vi "Check Modern MCP Request.vi"(7 "Mcp-Name":string, 8 "error in":errorcluster, 9 "Mcp-Method":string, 10 "protocol version":string, 11 "MCP Request Metadata":T1) -> (0 "error out":errorcluster, 1 "response":string, 2 "status code":u16, 3 "refused":bool)   [LabVIEW 2020, in "MCP Server.lvlib"]
doc: "Checks a request against the rules of MCP 2026-07-28 before it is handled, and says whether it is refused, with which HTTP status and which JSON-RPC error body. A legacy request is never refused here, except a JSON array that comes with modern headers.\n\nChecked in this order, the first failing check wins:\n- MCP-Protocol-Version header missing or different from the _meta protocolVersion: 400, -32020 (header mismatch).\n- protocolVersion not one of the modern versions of Supported Protocol Versions.vi: 400, -32022 with data.supported and data.requested.\n- Mcp-Method header missing or different from method: 400, -32020.\n- tools/call and prompts/get: Mcp-Name must equal params.name; resources/read: params.uri. A value =?base64?...?= is decoded first. Missing or different: 400, -32020.\n- io.modelcontextprotocol/clientCapabilities missing in params._meta: 400, -32602.\n- A method the modern era does not have (it has server/discover, tools/list, tools/call, prompts/list, prompts/get, resources/list, resources/read and resources/templates/list): 404, -32601. Notifications (no id) are not refused for this.\nA JSON array (batch) that comes with modern headers (an Mcp-Method header, or a modern MCP-Protocol-Version) is refused with 400, -32600.\n\nThe JSONtext errors are merged and cleared here. error in is passed through unchanged and does not stop the checks."
uses:
  MCP Server.lvlib
  5a72b263-2192-4f58-90a6-a4dd77c4a3e2.vi
  dc7c98e2-eea7-441a-9c60-934f37bda1c1.vi
  1b19c665-3783-46bd-b4e4-7a0e92e2d9d1.vi
  <vilib>/JDP Science/JSONtext/Variant to JSON Text.vi
  <vilib>/JDP Science/JSONtext/LVClass Serializer/JSONtext LVClass Serializer.lvclass
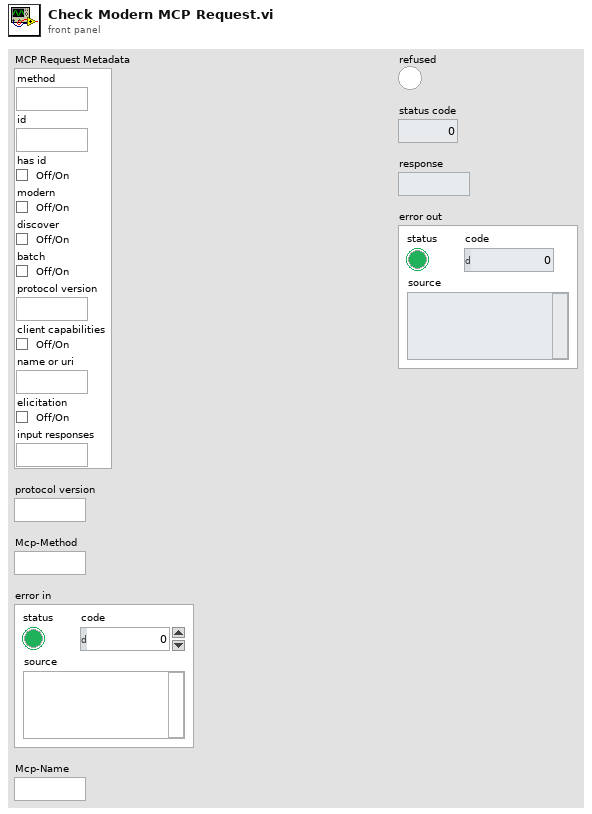
[diagram p1: front panel]
types:
  T1 = cluster{"method":string, "id":string, "has id":bool, "modern":bool, "discover":bool, "batch":bool, "protocol version":string, "client capabilities":bool, "name or uri":string, "elicitation":bool, "input responses":string}
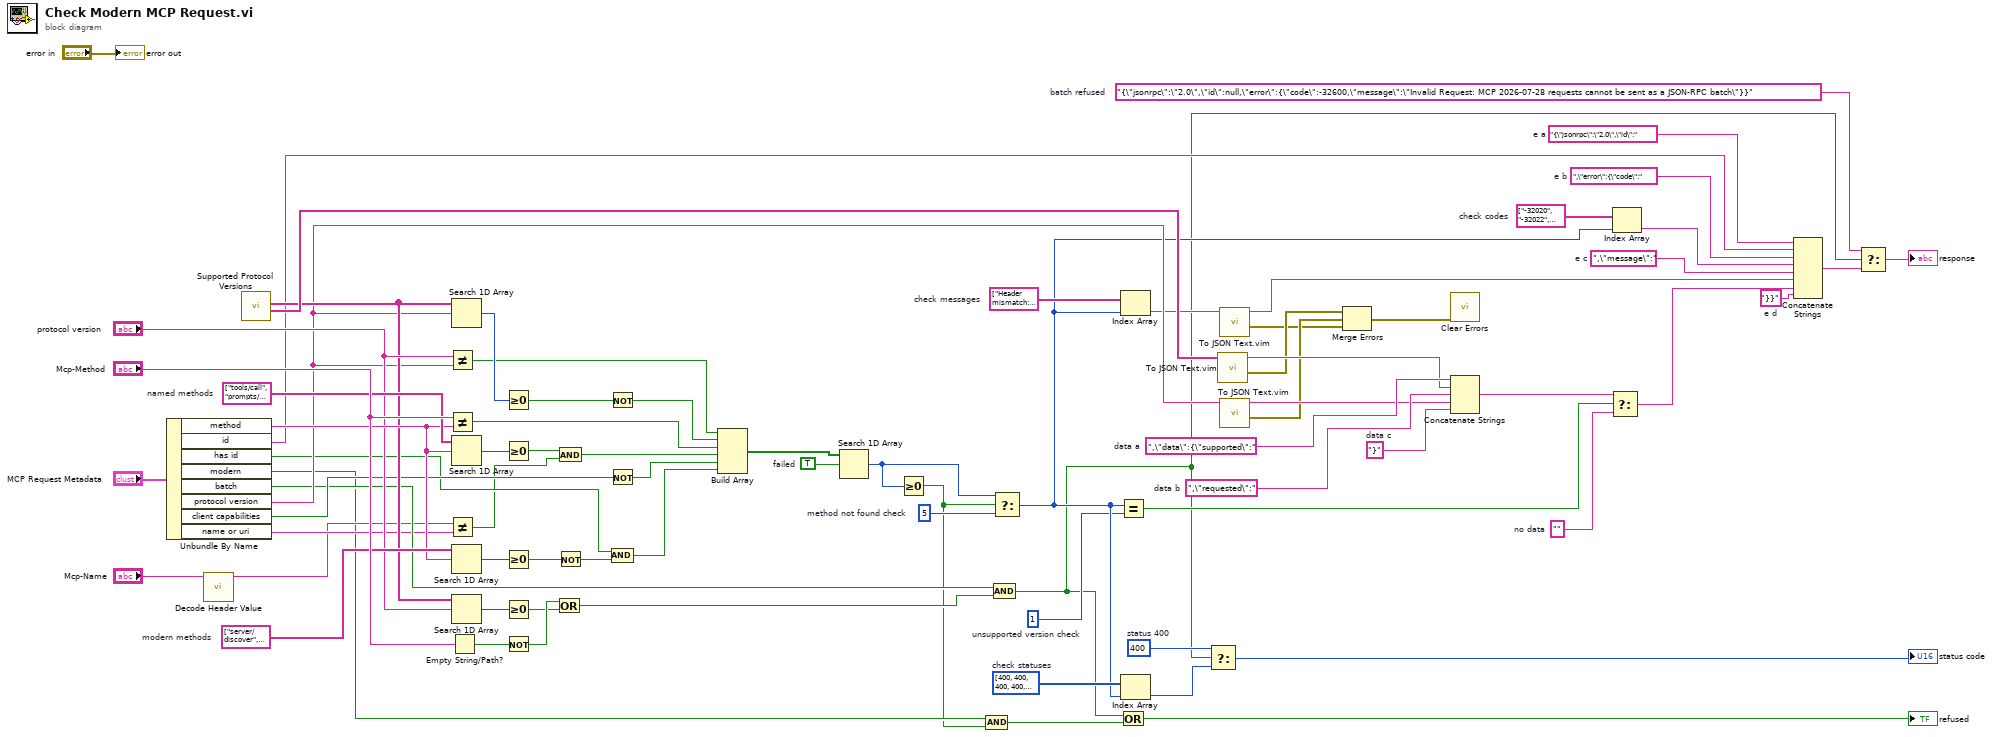
[diagram p0: block diagram]
diagram:
  w26 = 1  # unsupported version check
  w31 = 5  # method not found check
  w33 = TRUE  # failed
  w28 = u16[] [400, 400, 400, 400, 400, 404]  # check statuses
  w29 = string[] ["Header mismatch: the MCP-Protocol-Version header does not match params._meta io.modelcontextprotocol/protocolVersion", "Unsupported protocol version", "Header mismatch: the Mcp-Method header does not match method", "Header mismatch: the Mcp-Name header does not match params.name (params.uri for resources/read)", "Invalid params: params._meta io.modelcontextprotocol/clientCapabilities is required", "Method not found"]  # check messages
  w30 = string[] ["-32020", "-32022", "-32020", "-32020", "-32602", "-32601"]  # check codes
  w7 = u16 400  # status 400
  w9 = "{\"jsonrpc\":\"2.0\",\"id\":null,\"error\":{\"code\":-32600,\"message\":\"Invalid Request: MCP 2026-07-28 requests cannot be sent as a JSON-RPC batch\"}}"  # batch refused
  w13 = "}}"  # e d
  w16 = ",\"message\":"  # e c
  w18 = ",\"error\":{\"code\":"  # e b
  w20 = "{\"jsonrpc\":\"2.0\",\"id\":"  # e a
  w23 = ""  # no data
  w61 = "}"  # data c
  w63 = ",\"requested\":"  # data b
  w65 = ",\"data\":{\"supported\":"  # data a
  w72 = string[] ["server/discover", "tools/list", "tools/call", "prompts/list", "prompts/get", "resources/list", "resources/read", "resources/templates/list"]  # modern methods
  w73 = string[] ["tools/call", "prompts/get", "resources/read"]  # named methods
  n1 = Unbundle By Name("MCP Request Metadata") -> ("method"=w71:string, "id"=w19:string, "has id"=w57:bool, "modern"=w12:bool, "batch"=w59:bool, "protocol version"=w68:string, "client capabilities"=w67:bool, "name or uri"=w55:string)
  n2 = call "Decode Header Value.vi"("value"="Mcp-Name") -> ("decoded value"=w41:string)  [unwired: 10 in]
  n3 = call "Supported Protocol Versions.vi"() -> ("all versions"=w75:string[], "modern versions"=w69:string[])  [unwired: 9 in, 1 out]
  n4 = Not Equal?(x="protocol version", y=w68) -> (x != y?=w40:bool)
  n5 = Not Equal?(x="Mcp-Method", y=w71) -> (x != y?=w38:bool)
  n6 = Not Equal?(x=w41, y=w55) -> (x != y?=w54:bool)
  n7 = Empty String/Path?(string/path="Mcp-Method") -> (empty?=w66:bool)
  n8 = Search 1D Array(1D array=w69, element=w68) -> (index of element=w48:i32)  [unwired: 1 in]
  n9 = Search 1D Array(1D array=w73, element=w71) -> (index of element=w46:i32)  [unwired: 1 in]
  n10 = Search 1D Array(1D array=w72, element=w71) -> (index of element=w44:i32)  [unwired: 1 in]
  n11 = Search 1D Array(1D array=w69, element="protocol version") -> (index of element=w50:i32)  [unwired: 1 in]
  n12 = Greater Or Equal To 0?(x=w48) -> (x >= 0?=w47:bool)
  n13 = Greater Or Equal To 0?(x=w46) -> (x >= 0?=w45:bool)
  n14 = Greater Or Equal To 0?(x=w44) -> (x >= 0?=w43:bool)
  n15 = Greater Or Equal To 0?(x=w50) -> (x >= 0?=w49:bool)
  n16 = Not(x=w66) -> (.not. x?=w60:bool)
  n17 = Or(x=w60, y=w49) -> (x .or. y?=w58:bool)
  n18 = And(x=w45, y=w54) -> (x .and. y?=w37:bool)
  n19 = Not(x=w43) -> (.not. x?=w56:bool)
  n20 = Not(x=w47) -> (.not. x?=w39:bool)
  n21 = Not(x=w67) -> (.not. x?=w36:bool)
  n22 = And(x=w57, y=w56) -> (x .and. y?=w35:bool)
  n23 = Build Array(w40, w39, w38, w37, w36, w35) -> (w34:bool[])
  n24 = Search 1D Array(1D array=w34, element=w33) -> (index of element=w32:i32)  [unwired: 1 in]
  n25 = Greater Or Equal To 0?(x=w32) -> (x >= 0?=w11:bool)
  n26 = And(x=w12, y=w11) -> (x .and. y?=w10:bool)
  n27 = And(x=w59, y=w58) -> (x .and. y?=w6:bool)
  n28 = Select(t=w32, s=w11, f=w31) -> (s? t:f=w27:i32)
  n29 = Equal?(x=w27, y=w26) -> (x = y?=w24:bool)
  n30 = Or(x=w6, y=w10) -> (x .or. y?=→"refused":bool)
  n31 = Index Array(array=w29, index=w27) -> (element=w22:string)
  n32 = Index Array(array=w28, index=w27) -> (element=w5:u16)
  n33 = Select(t=w7, s=w6, f=w5) -> (s? t:f=→"status code":u16)
  n34 = call "To JSON Text.vim"("Anything"=w75) -> ("error out"=w53:errorcluster, "<JSON>"=w64:string)  [unwired: 9 in]
  n35 = call "To JSON Text.vim"("Anything"=w22) -> ("error out"=w21:errorcluster, "<JSON>"=w15:string)  [unwired: 9 in]
  n36 = call "To JSON Text.vim"("Anything"=w68) -> ("error out"=w52:errorcluster, "<JSON>"=w62:string)  [unwired: 9 in]
  n37 = Merge Errors(w53, w52, w21) -> (w51:errorcluster)
  n38 = call <vilib>:"Clear Errors.vi"("error in (no error)"=w51) -> ()  [unwired: 5 in, 2 out]
  n39 = Concatenate Strings(w65, w64, w63, w62, w61) -> (w25:string)
  n40 = Select(t=w25, s=w24, f=w23) -> (s? t:f=w14:string)
  n41 = Index Array(array=w30, index=w27) -> (element=w17:string)
  n42 = Concatenate Strings(w20, w19, w18, w17, w16, w15, w14, w13) -> (w8:string)
  n43 = Select(t=w9, s=w6, f=w8) -> (s? t:f=→"response":string)
  "error out" <- "error in"
